vi "test_Packet_SimpleTrackedTarget.vi"(8 "error in (no error)":errorcluster) -> (0 "error out":errorcluster, 3 "Test Passed":bool)   [LabVIEW 2019]
uses:
  <vilib>/Rock Robotics/WPI/ThirdParty/PhotonVisionLib/PhotonVisionLib.lvlib
  <vilib>/Rock Robotics/WPI/ThirdParty/JAS_Junk/TrajLib/Trajectory_Library.lvlib
  <vilib>/Rock Robotics/WPI/ThirdParty/PhotonVisionLib/TypeDef/TargetCornerType.ctl
  <vilib>/Rock Robotics/WPI/ThirdParty/PhotonVisionLib/TypeDef/PhotonTrackedTargetType.ctl
  <vilib>/Rock Robotics/WPI/ThirdParty/JAS_Junk/TrajLib/TypeDef/TRANSLATION3D.ctl
  <vilib>/Rock Robotics/WPI/ThirdParty/JAS_Junk/TrajLib/TypeDef/QUATERNION.ctl
  <vilib>/Rock Robotics/WPI/ThirdParty/JAS_Junk/TrajLib/TypeDef/ROTATION3D.ctl
  <vilib>/Rock Robotics/WPI/ThirdParty/JAS_Junk/TrajLib/TypeDef/TRANSFORM3D.ctl
panel:
  out "NextByte":i32
  out "size(s)":i32
  out "TrackedTarget 2":T1={"Yaw"=0.0, "Pitch"=0.0, "Area"=0.0, "Skew"=0.0, "MinAreaRectCorners"=[], "BestCameraToTarget"={"TRANSLATION3D"={"X"=0.0, "Y"=0.0, "Z"=0.0}, "ROTATION3D"={"Q_quaternion"={"R"=1.0, "V"=[0.0, 0.0, 0.0]}}, "XF"=FALSE}, "FiducialId"=0, "AltCameraToTarget"={"TRANSLATION3D"={"X"=0.0, "Y"=0.0, "Z"=0.0}, "ROTATION3D"={"Q_quaternion"={"R"=1.0, "V"=[0.0, 0.0, 0.0]}}, "XF"=FALSE}, "PoseAmbiguity"=0.0, "DetectedCorners"=[], "ObjDetectId"=0, "ObjDetectConf"=0.0} {"AltCameraToTarget"."TRANSLATION3D"."Z" format="%14.3f"; "AltCameraToTarget"."TRANSLATION3D"."Y" format="%14.3f"; "AltCameraToTarget"."TRANSLATION3D"."X" format="%14.3f"; "BestCameraToTarget"."TRANSLATION3D"."Z" format="%14.3f"; "BestCameraToTarget"."TRANSLATION3D"."Y" format="%14.3f"; "BestCameraToTarget"."TRANSLATION3D"."X" format="%14.3f"}
  out "TrackedTarget":T1={"Yaw"=0.0, "Pitch"=0.0, "Area"=0.0, "Skew"=0.0, "MinAreaRectCorners"=[], "BestCameraToTarget"={"TRANSLATION3D"={"X"=0.0, "Y"=0.0, "Z"=0.0}, "ROTATION3D"={"Q_quaternion"={"R"=1.0, "V"=[0.0, 0.0, 0.0]}}, "XF"=FALSE}, "FiducialId"=0, "AltCameraToTarget"={"TRANSLATION3D"={"X"=0.0, "Y"=0.0, "Z"=0.0}, "ROTATION3D"={"Q_quaternion"={"R"=1.0, "V"=[0.0, 0.0, 0.0]}}, "XF"=FALSE}, "PoseAmbiguity"=0.0, "DetectedCorners"=[], "ObjDetectId"=0, "ObjDetectConf"=0.0} {"AltCameraToTarget"."TRANSLATION3D"."Z" format="%14.3f"; "AltCameraToTarget"."TRANSLATION3D"."Y" format="%14.3f"; "AltCameraToTarget"."TRANSLATION3D"."X" format="%14.3f"; "BestCameraToTarget"."TRANSLATION3D"."Z" format="%14.3f"; "BestCameraToTarget"."TRANSLATION3D"."Y" format="%14.3f"; "BestCameraToTarget"."TRANSLATION3D"."X" format="%14.3f"}
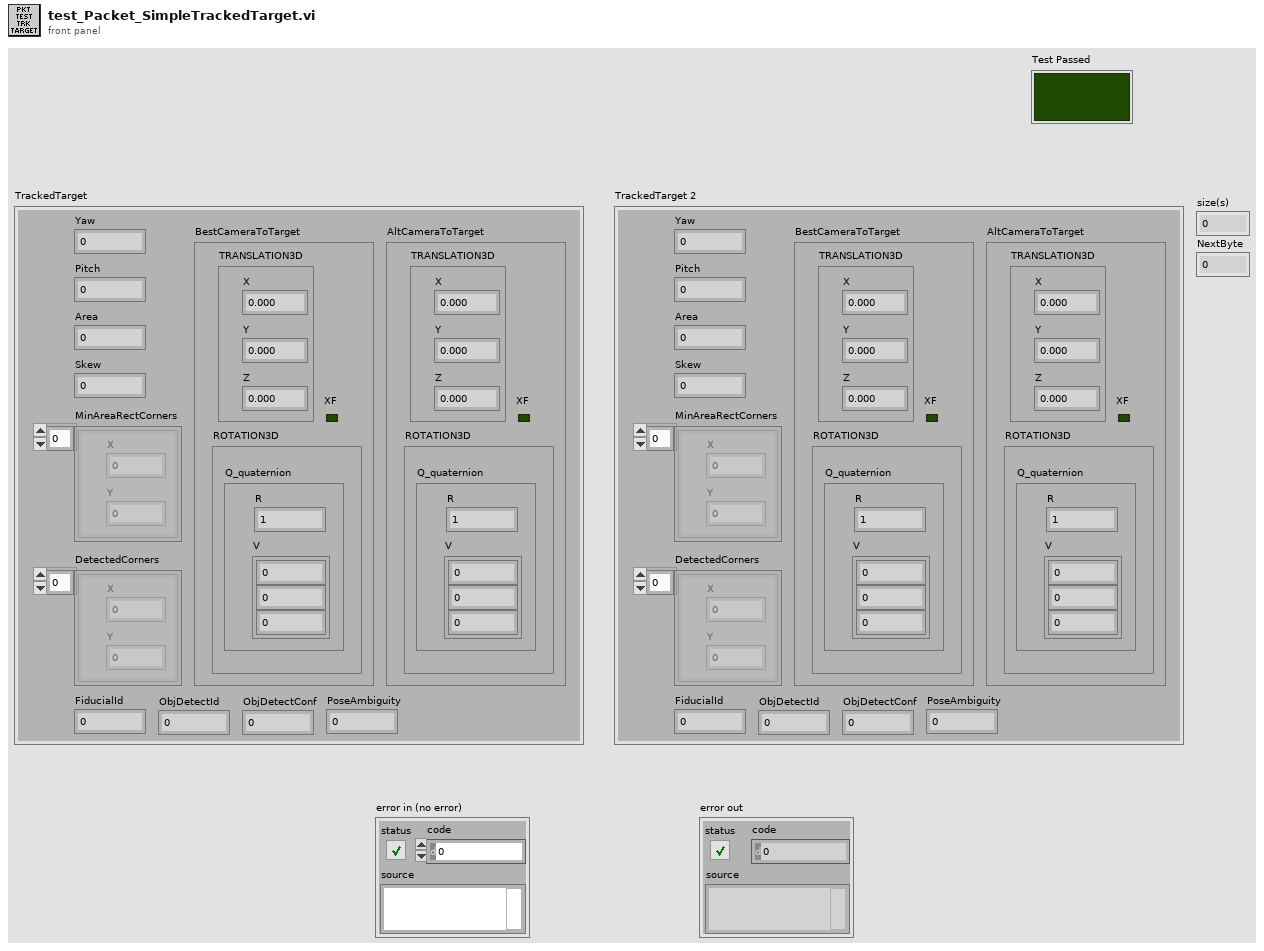
[diagram p1: front panel]
types:
  T1 = typedef "PhotonVisionLib.lvlib/PhotonTrackedTargetType.ctl" = cluster{"Yaw":dbl, "Pitch":dbl, "Area":dbl, "Skew":dbl, "MinAreaRectCorners":T2[], "BestCameraToTarget":T3, "FiducialId":i32, "AltCameraToTarget":T3, "PoseAmbiguity":dbl, "DetectedCorners":T2[], "ObjDetectId":i32, "ObjDetectConf":sgl}
  T2 = typedef "PhotonVisionLib.lvlib/TargetCornerType.ctl" = cluster{"X":dbl, "Y":dbl}
  T3 = typedef "Trajectory_Library.lvlib/TRANSFORM3D.ctl" = cluster{"TRANSLATION3D":T4, "ROTATION3D":T5, "XF":bool}
  T4 = typedef "Trajectory_Library.lvlib/TRANSLATION3D.ctl" = cluster{"X":dbl, "Y":dbl, "Z":dbl}
  T5 = typedef "Trajectory_Library.lvlib/ROTATION3D.ctl" = cluster{"Q_quaternion":T6}
  T6 = typedef "Trajectory_Library.lvlib/QUATERNION.ctl" = cluster{"R":dbl, "V":dbl[]}
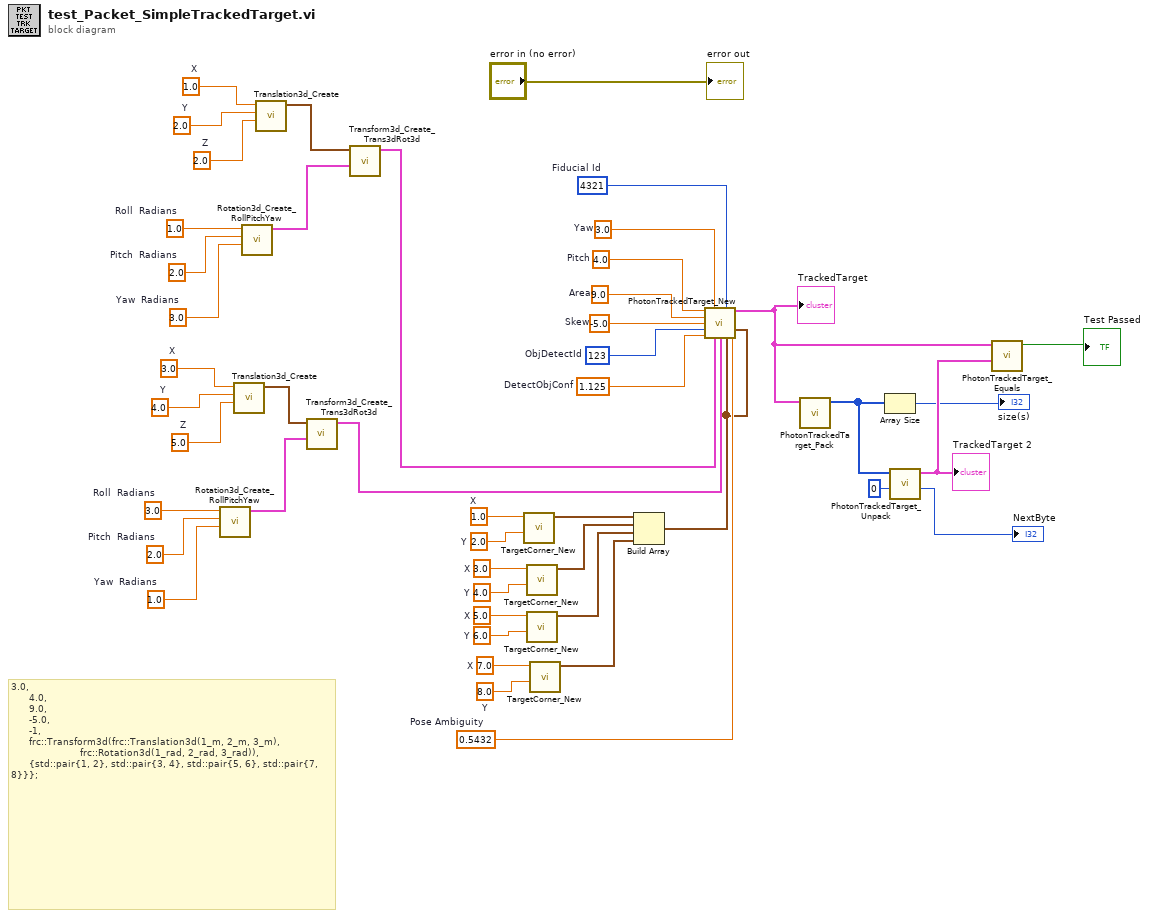
[diagram p0: block diagram]
diagram:
  w4 = sgl 1.125  # DetectObjConf
  w5 = 123  # ObjDetectId
  w11 = 7.0  # X
  w12 = 8.0  # Y
  w13 = 5.0  # X
  w14 = 6.0  # Y
  w15 = 3.0  # X
  w16 = 4.0  # Y
  w17 = 1.0  # X
  w18 = 2.0  # Y
  w24 = 3.0  # Roll  Radians
  w23 = 2.0  # Pitch  Radians
  w22 = 1.0  # Yaw  Radians
  w26 = 3.0  # X
  w27 = 4.0  # Y
  w28 = 5.0  # Z
  w33 = 1.0  # Roll  Radians
  w32 = 2.0  # Pitch  Radians
  w31 = 3.0  # Yaw  Radians
  w35 = 1.0  # X
  w36 = 2.0  # Y
  w37 = 2.0  # Z
  w38 = 0.5432  # Pose Ambiguity
  w39 = 4321  # Fiducial Id
  w43 = 4.0  # Pitch
  w44 = 9.0  # Area
  w45 = -5.0  # Skew
  w46 = 3.0  # Yaw
  # "3.0,\n      4.0,\n      9.0,\n      -5.0,\n      -1,\n      frc::Transform3d(frc::Translation3d(1_m, 2_m, 3_m),\n                       frc::Rotation3d(1_rad, 2_rad, 3_rad)),\n      {std::pair{1, 2}, std::pair{3, 4}, std::pair{5, 6}, std::pair{7, 8}}};"
  n1 = call <vilib>:"Rotation3d_Create_RollPitchYaw.vi"("Yaw"=w22, "Pitch"=w23, "Roll"=w24) -> ("Rotation3d"=w21:T5)  [unwired: 8 in]
  n2 = call <vilib>:"Translation3d_Create.vi"("Z"=w28, "Y"=w27, "X"=w26) -> ("TRANSLATION3D"=w25:T4)  [unwired: 8 in]
  n3 = call <vilib>:"Rotation3d_Create_RollPitchYaw.vi"("Yaw"=w31, "Pitch"=w32, "Roll"=w33) -> ("Rotation3d"=w30:T5)  [unwired: 8 in]
  n4 = call <vilib>:"Translation3d_Create.vi"("Z"=w37, "Y"=w36, "X"=w35) -> ("TRANSLATION3D"=w34:T4)  [unwired: 8 in]
  n5 = call <vilib>:"Transform3d_Create_Trans3dRot3d.vi"("Rotation3d"=w21, "Translation3d"=w25) -> ("Transform3d"=w20:T3)  [unwired: 9 in]
  n6 = call <vilib>:"Transform3d_Create_Trans3dRot3d.vi"("Rotation3d"=w30, "Translation3d"=w34) -> ("Transform3d"=w29:T3)  [unwired: 9 in]
  n7 = call <vilib>:"TargetCorner_New.vi"("Y"=w18, "X"=w17) -> ("TargetCorner"=w10:T2)  [unwired: 9 in]
  n8 = call <vilib>:"TargetCorner_New.vi"("Y"=w16, "X"=w15) -> ("TargetCorner"=w9:T2)  [unwired: 9 in]
  n9 = call <vilib>:"TargetCorner_New.vi"("Y"=w14, "X"=w13) -> ("TargetCorner"=w8:T2)  [unwired: 9 in]
  n10 = call <vilib>:"TargetCorner_New.vi"("Y"=w12, "X"=w11) -> ("TargetCorner"=w7:T2)  [unwired: 9 in]
  n11 = Build Array(w10, w9, w8, w7) -> (w6:T2[])
  n12 = call <vilib>:"PhotonTrackedTarget_New.vi"("Pitch"=w43, "Yaw"=w46, "Fiducial Id"=w39, "Area"=w44, "Skew"=w45, "ObjDetectId"=w5, "DetectedCorners"=w6, "DetectObjConf"=w4, "BestCameraToTarget"=w29, "AltCameraToTarget"=w20, "MinAreaRectCorners"=w6, "Pose Ambiguity"=w38) -> ("TrackedTarget"=w19:T1)  [unwired: 3 in]
  "TrackedTarget" <- w19
  n13 = call <vilib>:"PhotonTrackedTarget_Pack.vi"("TrackedTarget"=w19) -> ("RawData Out"=w3:u8[])  [unwired: 10 in]
  n14 = Array Size(array=w3) -> (size(s)=→"size(s)":i32)
  n15 = call <vilib>:"PhotonTrackedTarget_Unpack.vi"("StartByte"=0, "RawData"=w3) -> ("NextByte"=→"NextByte":i32, "TrackedTarget"=w41:T1)  [unwired: 8 in]
  "TrackedTarget 2" <- w41
  n16 = call <vilib>:"PhotonTrackedTarget_Equals.vi"("Other TrackedTarget"=w41, "TrackedTarget"=w19) -> ("Equals"=→"Test Passed":bool)  [unwired: 9 in]
  "error out" <- "error in (no error)"
